vi "Get Port.vi"(8 "error in (no error)":errorcluster caption="에러 입력(에러 없음)", 11 "RF Filter Box 입력":refnum<class "RF Filter Box.lvclass">) -> (0 "error out":errorcluster caption="에러 출력", 1 "Filter path":T1, 2 "Input path":T2, 3 "RF Filter Box 출력":refnum<class "RF Filter Box.lvclass">)   [LabVIEW 2023, in "RF Switch Box.lvlib" / "RF Filter Box.lvclass"]
uses:
  RF Filter Box.lvclass
  Type Definition/Input path.ctl
  RF Switch Box.lvlib
  Type Definition/Filter path.ctl
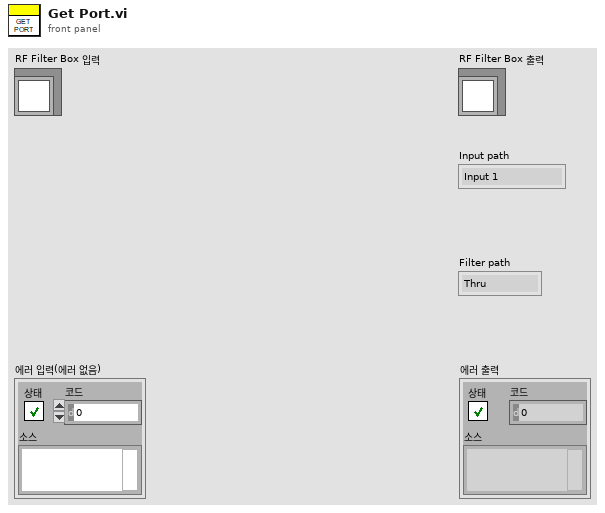
[diagram p1: front panel]
types:
  T1 = typedef "RF Switch Box.lvlib/Filter path.ctl" = enum16{"Thru", "Direct Amp", "1G HPF", "3G HPF", "7G HPF", "6G HPF", "port 1", "port 2", "port 3", "port 4", "port 5", "port 6", "port 7", "port 8", "port 9", "port 10", "port 11", "port 12", "port 13", "port 14", "port 15", "port 16", "port 17", "port 18"}
  T2 = typedef "RF Switch Box.lvlib/Input path.ctl" = enum16{"Input 1", "Input 2", "Input 3"}
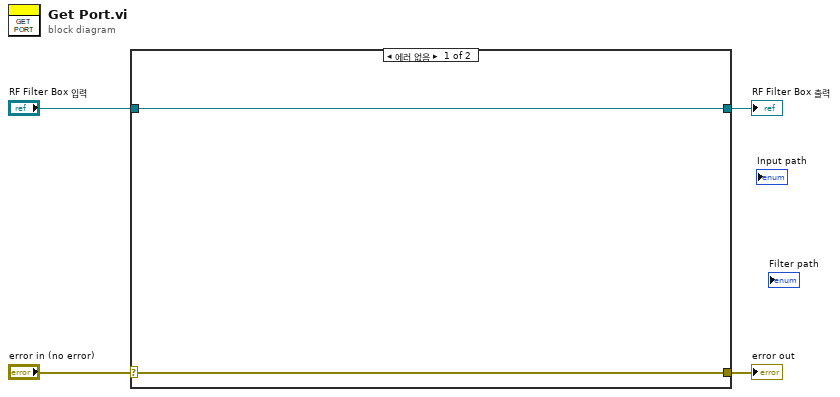
[diagram p0: block diagram]
diagram:
  n1 = case shown="에러 없음" "error in (no error)" {
    selector: "error in (no error)" -> [w5 w8]
    tunnel: [w5 w8] -> w3
    tunnel: [w6 w7] -> w1
    tunnel: "RF Filter Box 입력" -> [w6 w7]
    frame No Error {
    }
    frame Error {
    }
  }
  "error out" <- w3
  "RF Filter Box 출력" <- w1
